vi "LabVIEW VI code.vi"() -> ()   [LabVIEW 2026]
uses:
  <vilib>/DAQmx/read.llb/DAQmx Read (Analog 2D DBL NChan NSamp).vi
  <vilib>/Analysis/baseanly.llb/Mean (DBL).vi
  <vilib>/DAQmx/configure/timing.llb/DAQmx Timing (Sample Clock).vi
  <vilib>/DAQmx/miscellaneous.llb/DAQmx Fill In Error Info.vi
  <vilib>/Analysis/NI_AALBase.lvlib
panel:
  out "bytes written":i32
  out "String":string
  out "Array":string[](array[string])
  out "Waveform Chart":dbl[][](graph)
  in  "stop":bool
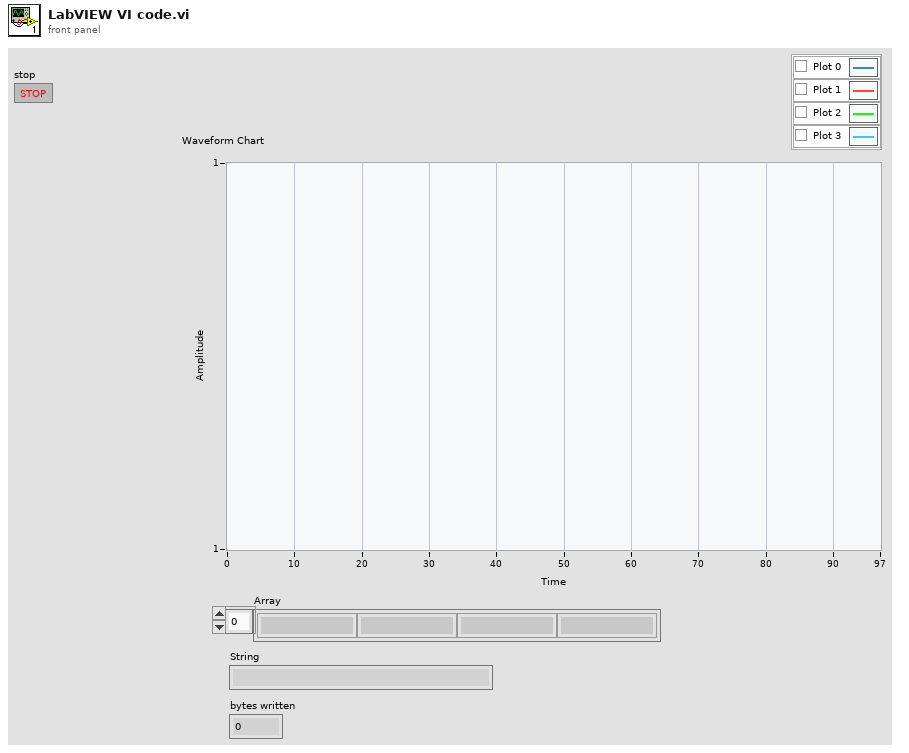
[diagram p1: front panel]
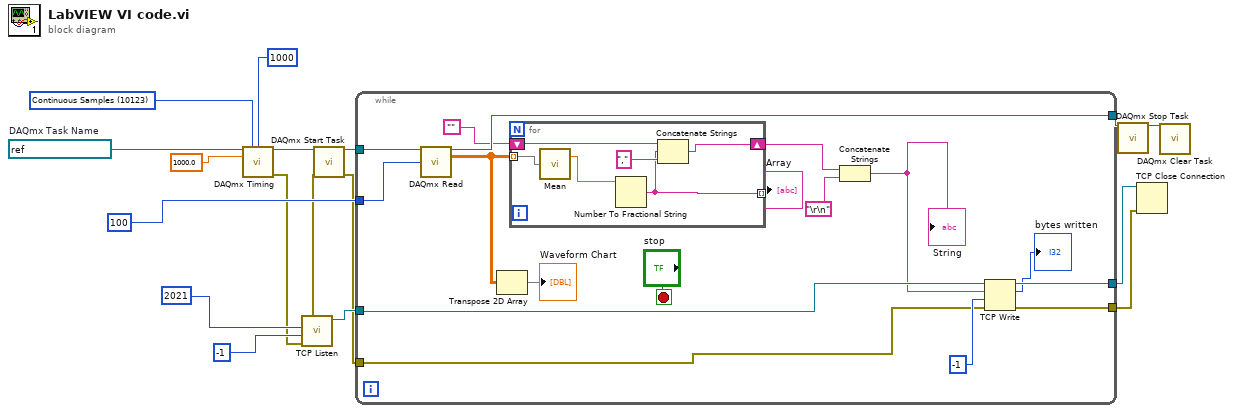
[diagram p0: block diagram]
diagram:
  w17 = 10123 items=["Finite Samples"=10178, "Continuous Samples"=10123, "Hardware Timed Single Point"=12522] ("sample mode")
  w12 = refnum<k21> "MyBridgeTask"  # DAQmx Task Name
  n1 = call-poly <vilib>:"DAQmx Timing.vi"("task/channels in"=w12, "sample mode"=w17, "samples per channel"=1000, "rate"=1000.0) -> ("task out"=w11:refnum<k21>, "error out"=w4:errorcluster)  [unwired: 10 in]
  n2 = call <vilib>:"TCP Listen.vi"("error in (no error)"=w4, "timeout ms (wait forever: -1)"=-1, "port"=2021) -> ("error out"=w2:errorcluster, "connection ID"=w5:refnum<k5>)  [unwired: 4 in, 3 out]
  n3 = call <vilib>:"DAQmx Start Task.vi"("task/channels in"=w11, "error in"=w2) -> ("task out"=w10:refnum<k21>, "error out"=w1:errorcluster)  [unwired: 12 in]
  n4 = while {
    tunnel: w10 -> [w33]
    tunnel: 100 ("samples per channel") -> [w32]
    tunnel: [w31] -> w14
    tunnel: w5 -> [w22]
    tunnel: [w26] -> w9
    tunnel: [w25] -> w8
    tunnel: w1 -> [w21]
    stop <- "stop" stop-if-true
    n5 = call-poly <vilib>:"DAQmx Read.vi"("task/channels in"=w33, "number of samples per channel"=w32) -> ("task out"=w31:refnum<k21>, "data"=w29:dbl[][])  [unwired: 11 in, 1 out]
    n6 = Transpose 2D Array(2D array=w29) -> (transposed array=→"Waveform Chart":dbl[][])
    n7 = for {
      tunnel: w29 -> [w40] mode=indexing
      tunnel: [w35] -> w28 mode=indexing
      shift-right: [w36] -> w19
      shift-left: "" -> [w38]
      n8 = call-poly <vilib>:"Mean.vi"("X"=w40) -> ("mean"=w39:dbl)  [unwired: 1 out]
      n9 = Number To Fractional String(number=w39) -> (F-format string=w35:string)  [unwired: 3 in]
      n10 = Concatenate Strings(w38, w35, "," ("string")) -> (w36:string)
    }
    "Array" <- w28
    n11 = Concatenate Strings(w19, "\r\n") -> (w20:string)
    "String" <- w20
    n12 = TCP Write(connection ID=w22, data in=w20, error in (no error)=w21, 9:-1) -> (connection ID out=w26:refnum<k5>, bytes written=→"bytes written":i32, error out=w25:errorcluster)
  }
  n13 = call <vilib>:"DAQmx Stop Task.vi"("task/channels in"=w14) -> ("task out"=w13:refnum<k21>)  [unwired: 13 in, 1 out]
  n14 = TCP Close Connection(connection ID=w9, error in (no error)=w8) -> ()  [unwired: 1 in, 2 out]
  n15 = call <vilib>:"DAQmx Clear Task.vi"("task in"=w13) -> ()  [unwired: 14 in, 1 out]
